vi "Tool_Unicode Update Tab Control Pages.vi"(5 "Interpret as Unicode (T)":bool=TRUE, 6 "error in (no error)":errorcluster, 7 "Page Captions":string[](array[string]), 9 "Tab Control":refnum<vi>) -> (0 "error out":errorcluster, 3 "Tab Control":refnum<vi>)   [LabVIEW 2019, in "Language Selection.lvlib"]
doc: "Uses \"Page Captions\" input array the rename TabControl's Page captions.\n- - -\nCopyright (c) 2026, Merecs Engineering GmbH"
uses:
  Language Selection.lvlib
  <vilib>/addons/Tools/Unicode/_subVIs/Convert ASCII to UTF-16LE (Scalar).vi
  <vilib>/addons/Tools/Unicode/UI Unicode Tools.lvlib
panel:
  # "Connector Pane"
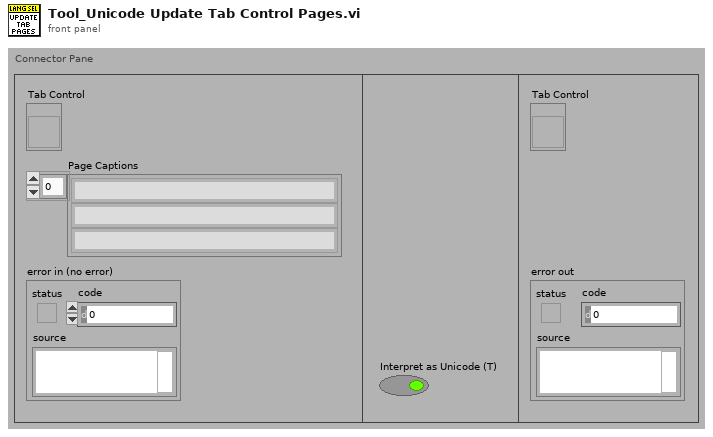
[diagram p1: front panel]
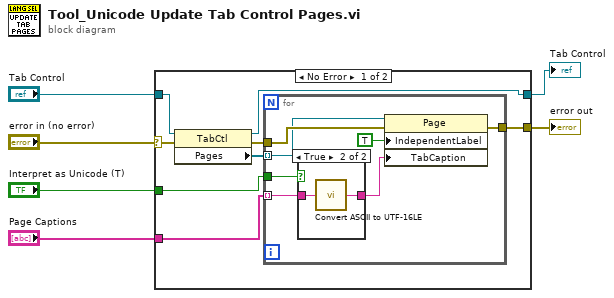
[diagram p0: block diagram]
diagram:
  n1 = case shown="No Error" "error in (no error)" {
    selector: "error in (no error)" -> [w9 w26]
    tunnel: [w14 w26] -> w6
    tunnel: "Page Captions" -> [w13 _]
    tunnel: "Tab Control" -> [w10 w25]
    tunnel: [w8 w25] -> w2
    tunnel: "Interpret as Unicode (T)" -> [w7 _]
    frame No Error {
      n2 = property class="TabCtl"(reference=w10, error in=w9) -> (reference out=w8:refnum<vi>, error out=w12:errorcluster, "Pages"=w11:refnum<vi>[])
      n3 = for {
        tunnel: w11 -> [w16] mode=indexing
        tunnel: w12 -> [w21]
        tunnel: w13 -> [w18] mode=indexing
        tunnel: [w19] -> w14
        tunnel: w7 -> [w15]
        n4 = case shown="True" w15 {
          tunnel: [w22 w23] -> w17
          tunnel: w18 -> [w22 w24]
          frame False {
          }
          frame True {
            n5 = call-poly <vilib>:"Convert ASCII to UTF-16LE.vi"("ASCII"=w24) -> ("Unicode"=w23:string)  [unwired: 4 in]
          }
        }
        n6 = property class="Page"(reference=w16, error in=w21, "IndependentLabel"=TRUE ("Independent Label"), "TabCaption"=w17) -> (error out=w19:errorcluster)  [unwired: 1 out]
      }
    }
    frame Error {
    }
  }
  "error out" <- w6
  "Tab Control" <- w2
